vi "Read Signals.vi"(8 "error in (no error)":errorcluster, 11 "session in":refnum<k21>) -> (0 "error out":errorcluster, 2 "session out":refnum<k21>, 3 "Array":T1[](array[typedef]))   [LabVIEW 2023]
uses:
  <resource>/objmgr/xnet.rc
  DUT Sample/typedefs/Signal Value.ctl
  <vilib>/xnet/xnet.llb/XNET Read (Signal Single-point).vi
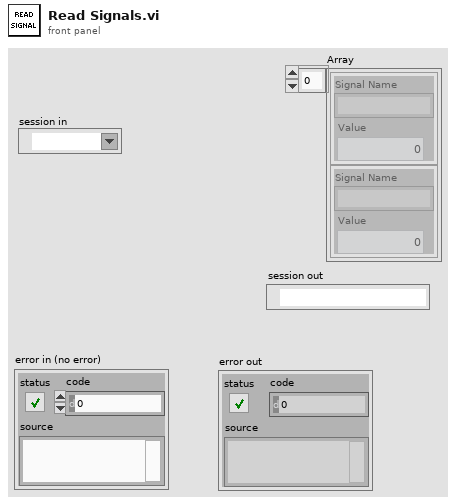
[diagram p1: front panel]
types:
  T1 = typedef "Signal Value.ctl" = cluster{"Signal Name":string, "Value":dbl}
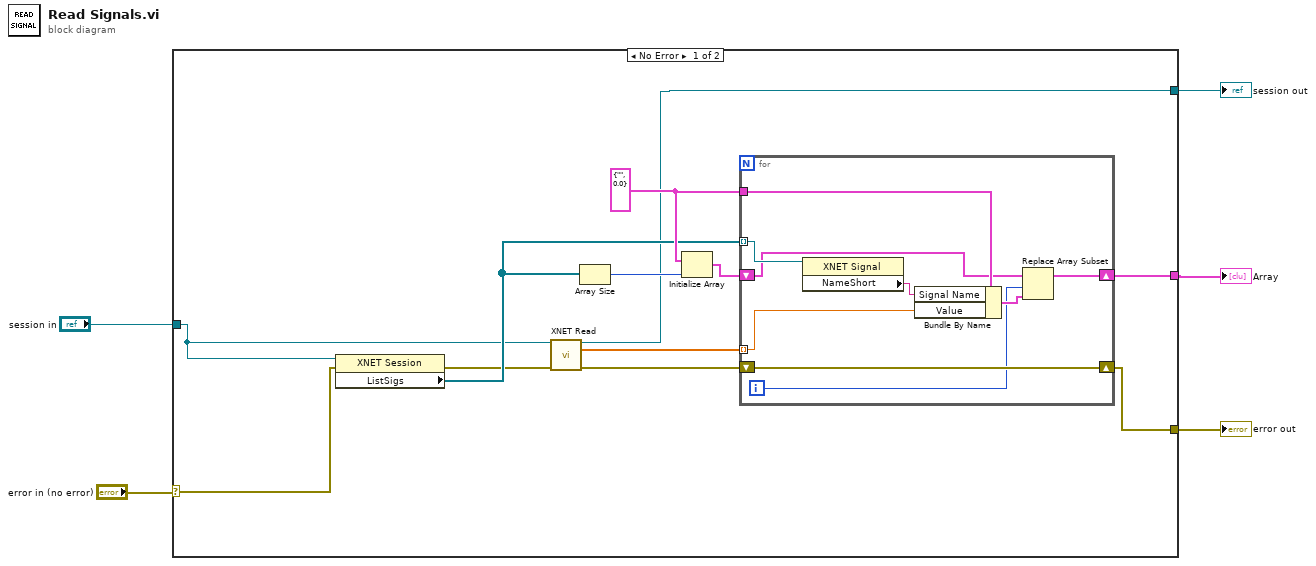
[diagram p0: block diagram]
diagram:
  n1 = case shown="No Error" "error in (no error)" {
    selector: "error in (no error)" -> [w7 w27]
    tunnel: [w12 _] -> w5
    tunnel: "session in" -> [w9 _]
    tunnel: [w8 w27] -> w2
    tunnel: [w6 _] -> w1
    frame No Error {
      w13 = T1 {"Signal Name"="", "Value"=0.0}
      n2 = property class="XNET Session"(reference=w9, error in=w7) -> (error out=w10:errorcluster, "ListSigs"=w11:refnum<k21>[])  [unwired: 1 out]
      n3 = call-poly <vilib>:"XNET Read.vi"("session in"=w9, "error in (no error)"=w10) -> ("session out"=w6:refnum<k21>, "data"=w17:dbl[], "error out"=w16:errorcluster)  [unwired: 11 in]
      n4 = Array Size(array=w11) -> (size(s)=w15:i32)
      n5 = Initialize Array(w13, w15) -> (w14:T1[])
      n6 = for {
        tunnel: w11 -> [w26] mode=indexing
        tunnel: w17 -> [w24] mode=indexing
        shift-right: [w21] -> w12
        shift-left: w14 -> [w22]
        tunnel: w13 -> [w25]
        shift-right: [w20] -> w8
        shift-left: w16 -> [w20]
        i -> [w18]
        n7 = property class="XNET Signal"(reference=w26) -> ("NameShort"=w23:string)  [unwired: 1 in, 2 out]
        n8 = Bundle By Name(cluster=w25, "Signal Name"=w23, "Value"=w24) -> (w19:T1)
        n9 = Replace Array Subset(array=w22, new element=w19, index=w18) -> (w21:T1[])
      }
    }
    frame Error {
    }
  }
  "error out" <- w2
  "Array" <- w5
  "session out" <- w1
